vi "[ce] Ticks counter (dataflow ready).vi"(5 "boolean in":bool, 6 "error in":errorcluster, 9 "ticks in":u32) -> (0 "error out":errorcluster, 1 "false":bool, 2 "true":bool=TRUE, 3 "ticks (current-input)":u32, 4 "dup boolean in":bool)   [LabVIEW 2021]
doc: "The VI returns value of the millisecond timer decreased by <B>ticks in</B>. If <B>ticks in</B> is zero, <B>ticks (current-input)</B> indicators contains the value of the millisecond timer; otherwise, returned value is a number of milliseconds elapsed since <B>ticks in</B> until this VI call.\n\n<B>boolean in</B> has no effect on VI execution, its value is returned in <B>dup boolean in</B> indicator.\n\n<B>false</B> indicator always returns FALSE. <B>true</B> indicator always returns TRUE. \n\n<B>error out</B> indicator returns the same values as <B>error in</B>\n\n::: CalcExpress Toolkit :::\nCopyright (c) 2000-2026 Konstantin Shifershteyn. All rights reserved."
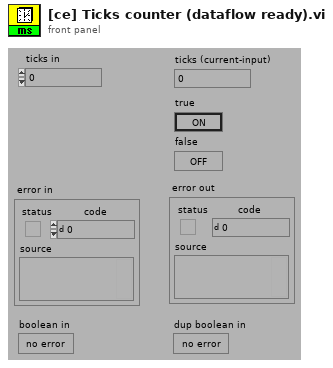
[diagram p1: front panel]
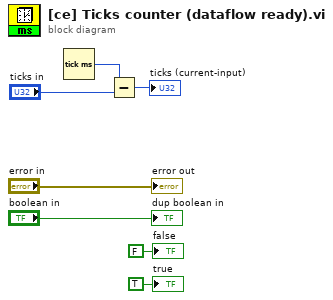
[diagram p0: block diagram]
diagram:
  n1 = Tick Count (ms)() -> (millisecond timer value=w6:u32)
  n2 = Subtract(x=w6, y="ticks in") -> (x-y=→"ticks (current-input)":u32)
  "error out" <- "error in"
  "true" <- TRUE ("true")
  "false" <- FALSE ("false")
  "dup boolean in" <- "boolean in"
